vi "Wire 3 terminal function.vi"(5 "Sink":refnum<vi>, 8 "error in (no error)":errorcluster, 9 "Source 2":refnum<vi>, 10 "Source 1":refnum<vi>, 11 "3 Terminal Function In":refnum<vi>) -> (0 "error out":errorcluster, 2 "Output Terminal":refnum<vi>, 3 "3 Terminal Function Out":refnum<vi>)   [LabVIEW 2012, in "Scripting Tools.lvlib"]
doc: "Wires up a 2 input, 1 output function, returning a reference to the output terminal as well."
uses:
  Scripting Tools.lvlib
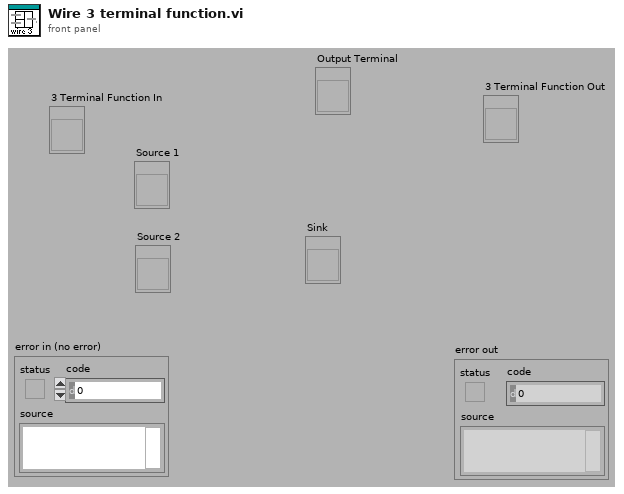
[diagram p1: front panel]
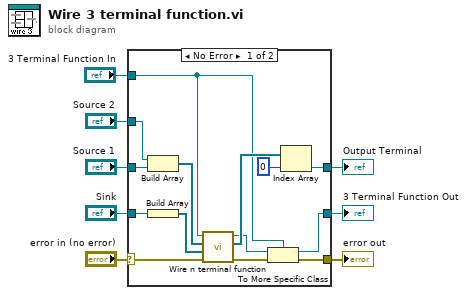
[diagram p0: block diagram]
diagram:
  n1 = case shown="No Error" "error in (no error)" {
    selector: "error in (no error)" -> [w11 w24]
    tunnel: [w9 w24] -> w8
    tunnel: "Sink" -> [w22 _]
    tunnel: "Source 1" -> [w20 _]
    tunnel: [w16 _] -> w5
    tunnel: "Source 2" -> [w15 _]
    tunnel: "3 Terminal Function In" -> [w14 w23]
    tunnel: [w13 w23] -> w2
    frame No Error {
      n2 = Build Array(w15, w20) -> (w19:refnum<vi>[])
      n3 = Build Array(w22) -> (w21:refnum<vi>[])
      n4 = call "Wire n terminal function.vi"("error in (no error)"=w11, "Sink Terminals"=w21, "Source Terminals"=w19, "Node In"=w14) -> ("error out"=w10:errorcluster, "Function Output Terminals"=w18:refnum<vi>[], "Node Out"=w12:refnum<vi>)  [unwired: 5 out]
      n5 = To More Specific Class(target class=w14, reference=w12, error in=w10) -> (specific class reference=w13:refnum<vi>, error out=w9:errorcluster)
      n6 = Index Array(array=w18, index=0) -> (element=w16:refnum<vi>)
    }
    frame Error {
    }
  }
  "3 Terminal Function Out" <- w2
  "error out" <- w8
  "Output Terminal" <- w5
